vi "SPI_Write_Byte_to_color_led_ws2813.vi"() -> ()   [LabVIEW 2020, in "CTI-Scratchpad.lvlib"]
uses:
  CTI-Scratchpad.lvlib
  CTI/SPI Config.ctl
  CTI/SPI Mode.ctl
  CTI/SPI Pins.ctl
  CTI/GPIO Number.ctl
  CTI/Session/Session.lvclass
  CTI/VisaComms/VisaComms.lvclass
  CTI/CTI.lvlib
panel:
  out "Led Color":u32(colorbox)=8094300
  out "B":u8
  out "G":u8
  out "R":u8
  out "error out":errorcluster
  in  "Color Box":u32(colorbox)=16711680
  in  "SPI Config":T1={"Mode"=0, "Data Bits"=32, "Pins"={"TX GPIO"=4, "RX GPIO"=7, "SCK GPIO"=2}}
  in  "Baud":u32=8000000 format="%.0p"
  in  "Bus":u8
  in  "Port":refnum<visa-resource-name>="COM5"
  # "SIG, Tx or MOSI on GPIO7  \nConnect the Grove connecteor on I2C1\nNo Switch lines"
  # "SIG, Tx or MOSI on GPIO19 (valid options: 3, 7, 19) \nConnect the Grove connecteor on D18\nSwitch lines white and yellow..."
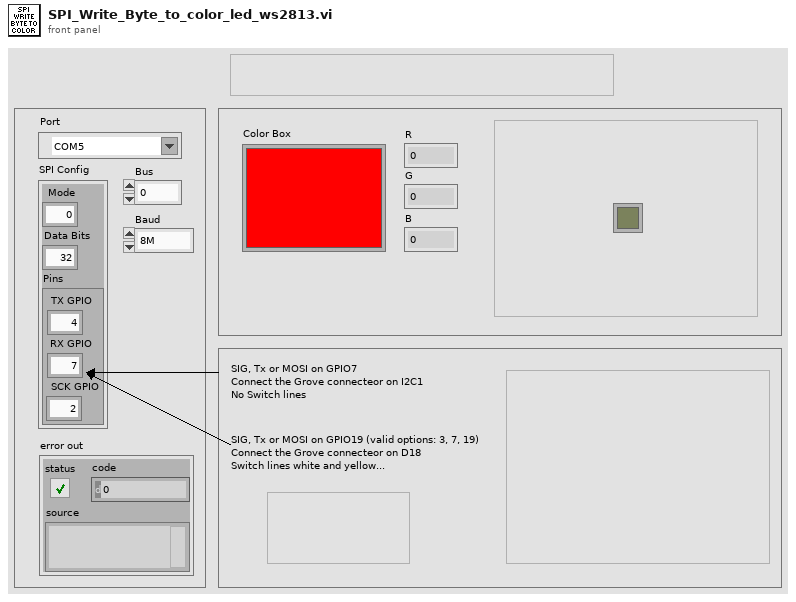
[diagram p1: front panel]
types:
  T1 = typedef "CTI.lvlib/SPI Config.ctl" = cluster{"Mode":T2, "Data Bits":i8, "Pins":T3}
  T2 = typedef "CTI.lvlib/SPI Mode.ctl" = i8
  T3 = typedef "CTI.lvlib/SPI Pins.ctl" = cluster{"TX GPIO":T4, "RX GPIO":T4, "SCK GPIO":T4}
  T4 = typedef "CTI.lvlib/GPIO Number.ctl" = i8
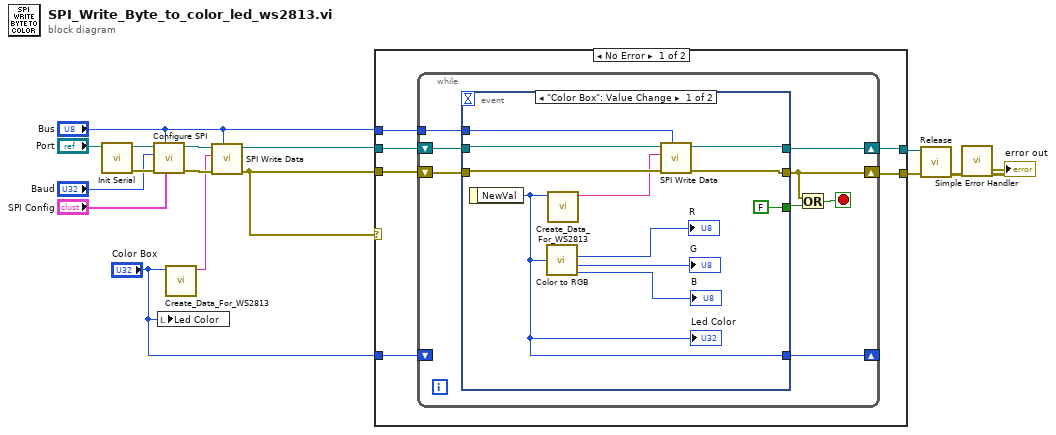
[diagram p0: block diagram]
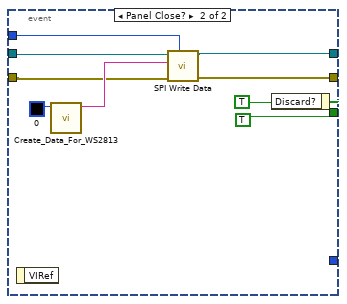
[diagram p2: hidden frame]
diagram:
  n1 = call "Init Serial.vi"("VISA resource name in"="Port") -> ("error out"=w15:errorcluster, "Session"=w14:refnum<class "Session.lvclass">)  [unwired: 8 in, 1 out]
  n2 = call "Configure SPI.vi"("SPI Config"="SPI Config", "SPI #"="Bus", "error in (no error)"=w15, "Baud"="Baud", "Session in"=w14) -> ("error out"=w6:errorcluster, "Session out"=w7:refnum<class "Session.lvclass">)  [unwired: 5 in]
  n3 = local write "Led Color"("Color Box") -> ()
  n4 = call "Create_Data_For_WS2813.vi"("Color Box"="Color Box") -> ("string"=w4:string)  [unwired: 10 in]
  n5 = call "SPI Write Data.vi"("SPI #"="Bus", "error in (no error)"=w6, "Data"=w4, "Session in"=w7) -> ("error out"=w3:errorcluster, "Session out"=w2:refnum<class "Session.lvclass">)  [unwired: 6 in]
  n6 = case shown="No Error" w3 {
    tunnel: [w18 w51] -> w11
    tunnel: [w17 w52] -> w10
    tunnel: w2 -> [w22 w51]
    tunnel: "Bus" -> [w21 _]
    tunnel: w3 -> [w20 w52]
    tunnel: "Color Box" -> [w19 _]
    frame No Error {
      n7 = while {
        tunnel: w21 -> [w27]
        shift-right: [w28] -> w18
        shift-left: w22 -> [w30]
        shift-right: [w25] -> w17
        shift-left: w20 -> [w29]
        shift-right: [w23] -> _
        shift-left: w19 -> [_]
        stop <- w24 stop-if-true
        n8 = event shown="[0] \"Color Box\": Value Change" {
          selector: _ -> [_ _]
          dyn-events: _ -> [_ _]
          timeout: _ -> [_ _]
          tunnel: w30 -> [w41 w46]
          tunnel: w29 -> [w40 w45]
          tunnel: [w31 w43] -> w25
          tunnel: [w32 w44] -> w28
          tunnel: w27 -> [w34 w42]
          tunnel: [FALSE TRUE ("Discard?")] -> w26
          tunnel: [w35 _] -> w23
          event "Color Box": Value Change {
            n9 = event-data() -> ("NewVal"=w35:u32)  [unwired: 1 in]
            "Led Color" <- w35
            n10 = call <vilib>:"Color to RGB.vi"("Color"=w35) -> ("R"=→"R":u8, "G"=→"G":u8, "B"=→"B":u8)  [unwired: 1 out]
            n11 = call "Create_Data_For_WS2813.vi"("Color Box"=w35) -> ("string"=w33:string)  [unwired: 10 in]
            n12 = call "SPI Write Data.vi"("SPI #"=w34, "error in (no error)"=w40, "Data"=w33, "Session in"=w41) -> ("error out"=w31:errorcluster, "Session out"=w32:refnum<class "Session.lvclass">)  [unwired: 6 in]
          }
          event Panel Close? {
            n13 = event-data() -> ()  [unwired: 1 in, 1 out]
            n14 = call "Create_Data_For_WS2813.vi"("Color Box"=u32 0) -> ("string"=w48:string)  [unwired: 10 in]
            n15 = call "SPI Write Data.vi"("SPI #"=w42, "error in (no error)"=w45, "Data"=w48, "Session in"=w46) -> ("error out"=w43:errorcluster, "Session out"=w44:refnum<class "Session.lvclass">)  [unwired: 6 in]
            n16 = event-data("Discard?"=TRUE) -> ()  [unwired: 1 in, 1 out]
          }
        }
        n17 = Or(x=w25, y=w26) -> (x .or. y?=w24:bool)
      }
    }
    frame Error {
    }
  }
  n18 = call-dynamic "Release.vi"("error in (no error)"=w10, "Session in"=w11) -> ("error out"=w8:errorcluster)  [unwired: 9 in]
  n19 = call <vilib>:"Simple Error Handler.vi"("error in (no error)"=w8) -> ("error out"=→"error out":errorcluster)  [unwired: 4 in, 4 out]
